vi "ROI_IN_Check.vi"(8 "도형Y좌표":dbl[](array[numeric]), 9 "도형X좌표":dbl[](array[numeric]), 10 "PCD_Y":i32[](array[numeric]), 11 "PCD_X":i32[](array[numeric])) -> (0 "논리적 OR":bool, 2 "ROI_IN_Y":dbl[](array[numeric]), 3 "ROI_IN_X":dbl[](array[numeric]))   [LabVIEW 2024]
uses:
  <vilib>/Analysis/geometry.llb/Point in Polygon (Scalar).vi
  <vilib>/Analysis/NI_AAL_Geometry.lvlib
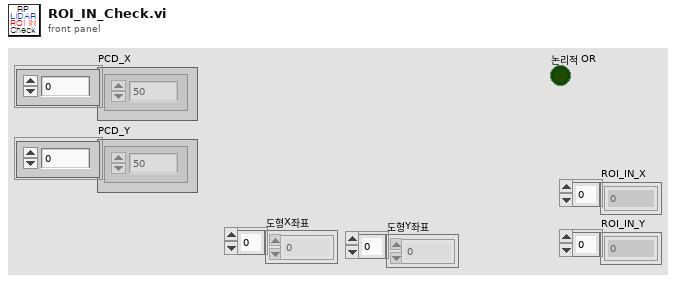
[diagram p1: front panel]
types:
  T1 = typedef "NI_AAL_Geometry.lvlib/Point in Polygon Position.ctl" = u16
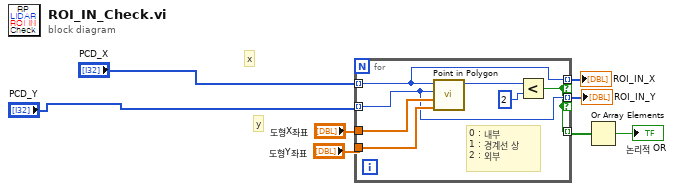
[diagram p0: block diagram]
diagram:
  # "y"
  # "x"
  n1 = for {
    tunnel: "PCD_Y" -> [w10] mode=indexing
    tunnel: "PCD_X" -> [w11] mode=indexing
    tunnel: "도형X좌표" -> [w15]
    tunnel: "도형Y좌표" -> [w14]
    tunnel: [w11] -> w6 mode=indexing if=w9
    tunnel: [w10] -> w5 mode=indexing if=w9
    tunnel: [w9] -> w4 mode=indexing
    # "0 : 내부\n1 : 경계선 상\n2 : 외부"
    n2 = call-poly <vilib>:"Point in Polygon.vi"("Polygon Y"=w14, "Polygon X"=w15, "y"=w10, "x"=w11) -> ("position"=w13:T1)  [unwired: 6 in, 1 out]
    n3 = Less?(x=w13, y=u16 2) -> (x < y?=w9:bool)
  }
  "ROI_IN_X" <- w6
  "ROI_IN_Y" <- w5
  n4 = Or Array Elements(Boolean array=w4) -> (logical OR=→"논리적 OR":bool)
